vi "Starting.vi"(4 "Async Elements":refnum<class "Async Elements.lvclass">, 6 "VI Ref":refnum<vi>, 7 "Actor in":refnum<class "Actor.lvclass">, 10 "Refs":refnum<class "Refs.lvclass">) -> (0 "Error out":errorcluster, 2 "Address":refnum<data-value>, 5 "Actor out":refnum<class "Actor.lvclass">)   [LabVIEW 2020, in "jettl.lvlib" / "Notifier Transport.lvlib"]
uses:
  Notifier Transport.lvlib
  Actor/Actor.lvclass
  Refs/Refs.lvclass
  Msg/Msg.lvclass
  Async Elements/Async Elements.lvclass
  Base Async Elements/Base Async Elements/Base Async Elements.lvclass/Base Async Elements.ctl
  Base Attributes/Base Attributes/Base Attributes.lvclass/Base Attributes.ctl
  Notifier Transport/Notifier Transport.lvclass/Notifier Transport.ctl
  Update Attributes A.vi
  Update Attributes B.vi
  Base Async Elements/Read Async Elements.vi
  Base Attributes/Init Attributes.vi
  Base Async Elements/Base Async Elements/Read Async Elements.vi
  Base Attributes/Base Attributes/Init Attributes.vi
  Notifier Transport/Notifier Transport.lvclass
  C:/git/jettl/src/jettl/jettl/Transport/Transport.lvclass
  Base Attributes/Base Attributes/Base Attributes.lvclass
  C:/git/jettl/src/jettl/jettl/Attributes/Attributes.lvclass
  Attributes/Attributes.lvclass
  Base Async Elements/Base Async Elements/Base Async Elements.lvclass
  Transport/Transport.lvclass
  jettl.lvlib
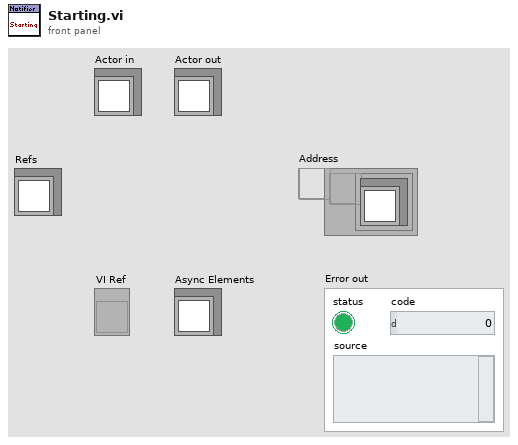
[diagram p1: front panel]
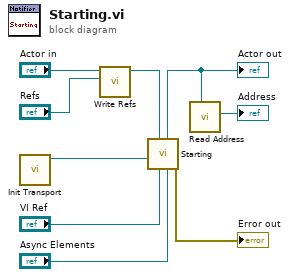
[diagram p0: block diagram]
diagram:
  n1 = call "Init Transport.vi"() -> ("Notifier Transport out"=w1:refnum<class "Notifier Transport.lvclass">)  [unwired: 11 in]
  n2 = call-dynamic "Write Refs.vi"("Refs"="Refs", "Actor in"="Actor in") -> ("Actor out"=w7:refnum<class "Actor.lvclass">)  [unwired: 9 in]
  n3 = call "Starting.vi"("Async Elements"="Async Elements", "VI Ref"="VI Ref", "Actor in"=w7, "Transport"=w1) -> ("Error out"=→"Error out":errorcluster, "Actor out"=w5:refnum<class "Actor.lvclass">)  [unwired: 6 in]
  "Actor out" <- w5
  n4 = call "Read Address.vi"("Actor"=w5) -> ("Address"=→"Address":refnum<data-value>)  [unwired: 10 in]
